vi "Instantiate.vi"(0 "projectspecificscripmanager in":refnum<class "projectspecificscripmanager.lvclass">, 5 "Output Terminal":refnum<class "Output Terminal.lvclass">, 7 "RT Variables":refnum<class "RT Variables.lvclass">, 9 "Function Directory[]":path[](array[path]), 11 "error in (no error)":errorcluster) -> (4 "projectspecificscripmanager out":refnum<class "projectspecificscripmanager.lvclass">, 15 "error out":errorcluster)   [LabVIEW 2020, in "projectspecificscripmanager.lvclass"]
uses:
  projectspecificscripmanager.lvclass
  source code/LSL components/output terminal/Base/Output Terminal.lvclass
  source code/LSL components/variables/RT Variables/RT Variables.lvclass
  source code/LSL components/functions/functions list/Statement/Statement.lvclass
  D:/petwork/LabVIEW-Script-Language/source code/LSL components/functions/functionsbase/functionbase.lvclass
  source code/LSL components/functions/functions list/UI Functions/UI Functions.lvclass
  source code/LSL components/functions/functions list/Array Functions/Array Functions.lvclass
  source code/LSL components/functions/functions list/Bitwise Functions/Bitwise Functions.lvclass
  source code/LSL components/functions/functions list/Boolean Functions/Boolean Functions.lvclass
  source code/LSL components/functions/functions list/Comparison Functions/Comparison Functions.lvclass
  source code/LSL components/functions/functions list/Numeric Functions/Numeric Functions.lvclass
  source code/LSL components/functions/functions list/String Functions/String Functions.lvclass
  source code/LSL components/functions/functions list/Structure If Else/Structure If Else.lvclass
  source code/LSL components/functions/functions list/Structure Loop/Structure Loop.lvclass
  source code/LSL components/functions/functions list/Timing Functions/Timing Functions.lvclass
  source code/LSL components/scripts/scripts manager/scripts manager.lvclass
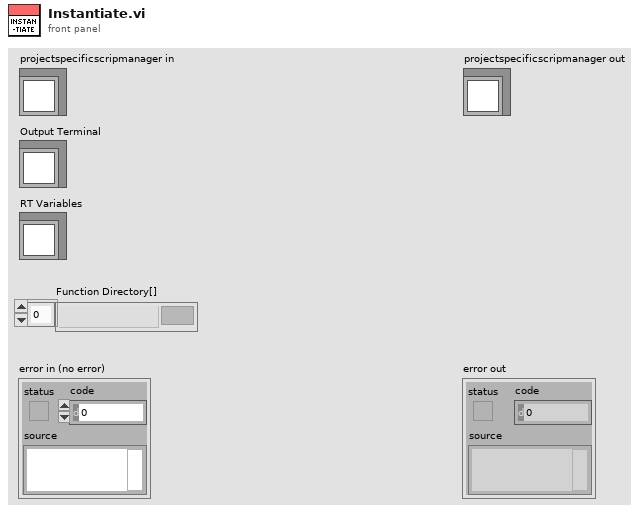
[diagram p1: front panel]
types:
  T1 = cluster{"String":string, "Comparison Functions.lvclass":refnum<class "Comparison Functions.lvclass">}
  T2 = cluster{"String":string, "Structure If Else.lvclass":refnum<class "Structure If Else.lvclass">}
  T3 = cluster{"String":string, "Timing Functions.lvclass":refnum<class "Timing Functions.lvclass">}
  T4 = cluster{"String":string, "Array Functions.lvclass":refnum<class "Array Functions.lvclass">}
  T5 = cluster{"String":string, "Boolean Functions.lvclass":refnum<class "Boolean Functions.lvclass">}
  T6 = cluster{"String":string, "String Functions.lvclass":refnum<class "String Functions.lvclass">}
  T7 = cluster{"String":string, "Structure Loop.lvclass":refnum<class "Structure Loop.lvclass">}
  T8 = cluster{"String":string, "UI Functions.lvclass":refnum<class "UI Functions.lvclass">}
  T9 = cluster{"String":string, "Statement.lvclass":refnum<class "Statement.lvclass">}
  T10 = cluster{"String":string, "Bitwise Functions.lvclass":refnum<class "Bitwise Functions.lvclass">}
  T11 = cluster{"String":string, "Numeric Functions.lvclass":refnum<class "Numeric Functions.lvclass">}
  T12 = cluster{"String":string, "UI Functions.lvclass":refnum<class "functionbase.lvclass">}[]
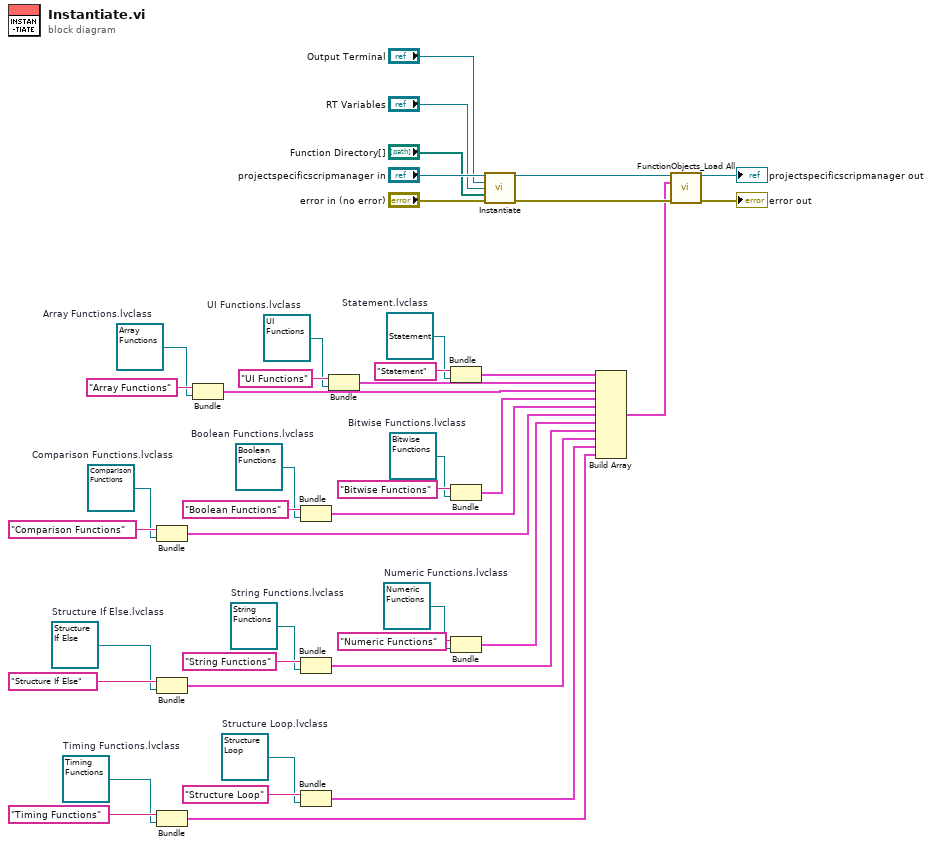
[diagram p0: block diagram]
diagram:
  w7 = refnum<class "Timing Functions.lvclass"> refnum  # Timing Functions.lvclass
  w8 = refnum<class "Structure Loop.lvclass"> refnum  # Structure Loop.lvclass
  w9 = refnum<class "Structure If Else.lvclass"> refnum  # Structure If Else.lvclass
  w10 = refnum<class "String Functions.lvclass"> refnum  # String Functions.lvclass
  w11 = refnum<class "Numeric Functions.lvclass"> refnum  # Numeric Functions.lvclass
  w20 = refnum<class "Comparison Functions.lvclass"> refnum  # Comparison Functions.lvclass
  w21 = refnum<class "Boolean Functions.lvclass"> refnum  # Boolean Functions.lvclass
  w22 = refnum<class "Bitwise Functions.lvclass"> refnum  # Bitwise Functions.lvclass
  w26 = refnum<class "Array Functions.lvclass"> refnum  # Array Functions.lvclass
  w30 = refnum<class "UI Functions.lvclass"> refnum  # UI Functions.lvclass
  w32 = refnum<class "Statement.lvclass"> refnum  # Statement.lvclass
  n1 = Bundle("String"="Comparison Functions", "Comparison Functions.lvclass"=w20) -> (w17:T1)  [unwired: 1 in]
  n2 = Bundle("String"="Structure If Else", "Structure If Else.lvclass"=w9) -> (w4:T2)  [unwired: 1 in]
  n3 = Bundle("String"="Timing Functions", "Timing Functions.lvclass"=w7) -> (w2:T3)  [unwired: 1 in]
  n4 = Bundle("String"="Array Functions", "Array Functions.lvclass"=w26) -> (w27:T4)  [unwired: 1 in]
  n5 = Bundle("String"="Boolean Functions", "Boolean Functions.lvclass"=w21) -> (w18:T5)  [unwired: 1 in]
  n6 = Bundle("String"="String Functions", "String Functions.lvclass"=w10) -> (w5:T6)  [unwired: 1 in]
  n7 = Bundle("String"="Structure Loop", "Structure Loop.lvclass"=w8) -> (w3:T7)  [unwired: 1 in]
  n8 = Bundle("String"="UI Functions", "UI Functions.lvclass"=w30) -> (w29:T8)  [unwired: 1 in]
  n9 = Bundle("String"="Statement", "Statement.lvclass"=w32) -> (w34:T9)  [unwired: 1 in]
  n10 = Bundle("String"="Bitwise Functions", "Bitwise Functions.lvclass"=w22) -> (w19:T10)  [unwired: 1 in]
  n11 = Bundle("String"="Numeric Functions", "Numeric Functions.lvclass"=w11) -> (w6:T11)  [unwired: 1 in]
  n12 = call-parent "Instantiate.vi"("scripts manager in"="projectspecificscripmanager in", "Output Terminal"="Output Terminal", "RT Variables"="RT Variables", "Function Directory[]"="Function Directory[]", "error in (no error)"="error in (no error)") -> ("scripts manager out"=w37:refnum<class "projectspecificscripmanager.lvclass">, "error out"=w38:errorcluster)  [unwired: 9 in]
  n13 = Build Array(w34, w29, w27, w19, w18, w17, w6, w5, w4, w3, w2) -> (w1:T12)
  n14 = call-dynamic "FunctionObjects_Load All.vi"("scripts manager in"=w37, "Function Objects In"=w1, "error in (no error)"=w38) -> ("scripts manager out"=→"projectspecificscripmanager out":refnum<class "projectspecificscripmanager.lvclass">, "error out"=→"error out":errorcluster)  [unwired: 11 in]
